vi "Set Device Parameters.vi"(8 "error in":errorcluster, 10 "device parameters":T1 {"coupling mode" items=["API429_CHANNEL_COUPLING_EXT", "API429_CHANNEL_COUPLING_DUAL", "API429_CHANNEL_COUPLING_INT"]}, 11 "custom device":T2=18446744073709551615 format="%.0x") -> (0 "error out":errorcluster, 3 "custom device ref out":T2 format="%.0x")   [LabVIEW 2020, in "AIM ARINC 429 Scripting.lvlib"]
doc: "Specifies AIM hardware device parameters such as <b>pxi slot</b>."
uses:
  AIM ARINC 429 Scripting.lvlib
  <vilib>/NI VeriStand/Custom Device API/Custom Device Item Ref.ctl
  Shared/Device Parameters.ctl
  Constants.vi
  <vilib>/NI VeriStand/Custom Device API/Set Item Property (I32).vi
  <vilib>/NI VeriStand/Custom Device API/Custom Device API.lvlib
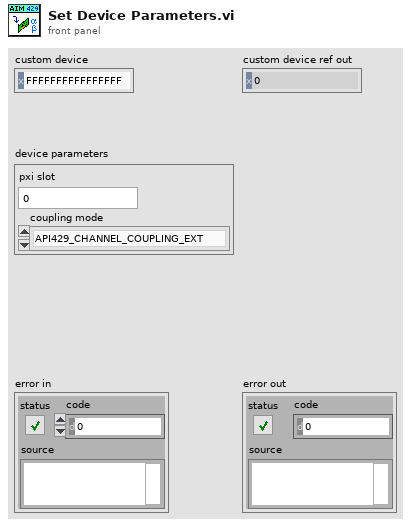
[diagram p1: front panel]
types:
  T1 = typedef "Device Parameters.ctl" = cluster{"pxi slot":u8, "coupling mode":u32}
  T2 = typedef "Custom Device API.lvlib/Custom Device Item Ref.ctl" = u64
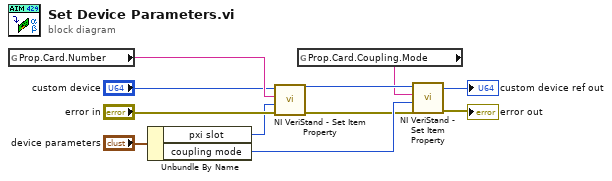
[diagram p0: block diagram]
diagram:
  n1 = global read "Constants.vi" "Prop.Card.Number"() -> (w11:string)
  n2 = Unbundle By Name("device parameters") -> ("pxi slot"=w7:u8, "coupling mode"=w6:u32)
  n3 = call-poly <vilib>:"NI VeriStand - Set Item Property.vi"("error in (no error)"="error in", "Value"=w7, "Property Name"=w11, "Item Ref in"="custom device") -> ("error out"=w4:errorcluster, "Item Ref out"=w5:T2)  [unwired: 5 in, 1 out]
  n4 = global read "Constants.vi" "Prop.Card.Coupling.Mode"() -> (w1:string)
  n5 = call-poly <vilib>:"NI VeriStand - Set Item Property.vi"("error in (no error)"=w4, "Value"=w6, "Property Name"=w1, "Item Ref in"=w5) -> ("error out"=→"error out":errorcluster, "Item Ref out"=→"custom device ref out":T2)  [unwired: 5 in, 1 out]
